vi "libssh2_session_get_blocking.vi"(8 "error in (no error)":errorcluster, 11 "session":T1) -> (0 "error out":errorcluster, 2 "blocking":bool)   [LabVIEW 2017, in "libssh2.lvlib"]
doc: "Get the blocking mode for a session."
uses:
  libssh2.lvlib
  Session Refnum.ctl
  Not A Session.vi
  <vilib>/Utility/error.llb/Error Cluster From Error Code.vi
  Global Settings.vi
  Read Session Refnum.vi
  <vilib>/Utility/semaphor.llb/Acquire Semaphore.vi
  <vilib>/Utility/semaphor.llb/Release Semaphore.vi
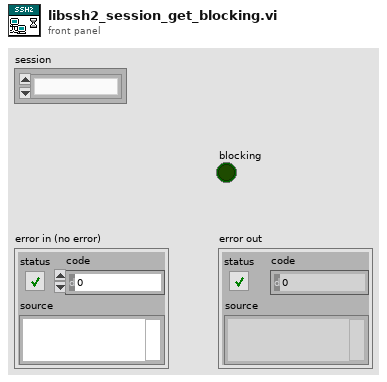
[diagram p1: front panel]
types:
  T1 = typedef "libssh2.lvlib/Session Refnum.ctl" = refnum<k1>
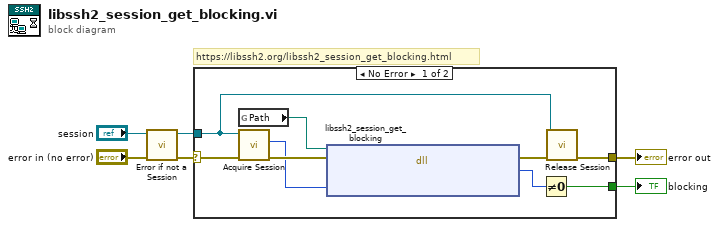
[diagram p0: block diagram]
diagram:
  # "https://libssh2.org/libssh2_session_get_blocking.html"
  n1 = call "Error if not a Session.vi"("error in (no error)"="error in (no error)", "session"="session") -> ("error out"=w3:errorcluster, "session out"=w1:T1)  [unwired: 8 in]
  n2 = case shown="No Error" w3 {
    selector: w3 -> [w14 w16]
    tunnel: [w8 w16] -> w6
    tunnel: w1 -> [w7 _]
    tunnel: [w13 _] -> w4
    frame No Error {
      n3 = global read "Global Settings.vi" "Path"() -> (w10:path)
      n4 = call "Acquire Session.vi"("error in (no error)"=w14, "session"=w7) -> ("error out"=w12:errorcluster, "LIBSSH2_SESSION*"=w11:u64)  [unwired: 7 in, 1 out]
      n5 = dll-call lib="?" fn="libssh2_session_get_blocking"(path in=w10, error in=w12, "session"=w11) -> (error out=w15:errorcluster, "return value"=w9:i32)  [unwired: 2 in, 1 out]
      n6 = Not Equal To 0?(x=w9) -> (x != 0?=w13:bool)
      n7 = call "Release Session.vi"("error in (no error)"=w15, "session"=w7) -> ("error out"=w8:errorcluster)  [unwired: 9 in]
    }
    frame Error {
    }
  }
  "error out" <- w6
  "blocking" <- w4
